vi "Set Result Configuration.vi"(11 "error in (no error)":errorcluster) -> (15 "error out":errorcluster)   [LabVIEW 2021, in "Voltage Measurement.lvlib"]
uses:
  09223ba7-b474-4af4-80b2-5f8b06bdc601.vi
  <vilib>/JDP Science/JSONtext/Variant to JSON Text.vi
  <vilib>/JDP Science/JSONtext/LVClass Serializer/JSONtext LVClass Serializer.lvclass
  Voltage Measurement.lvlib
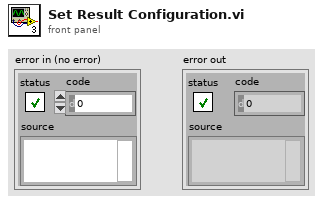
[diagram p1: front panel]
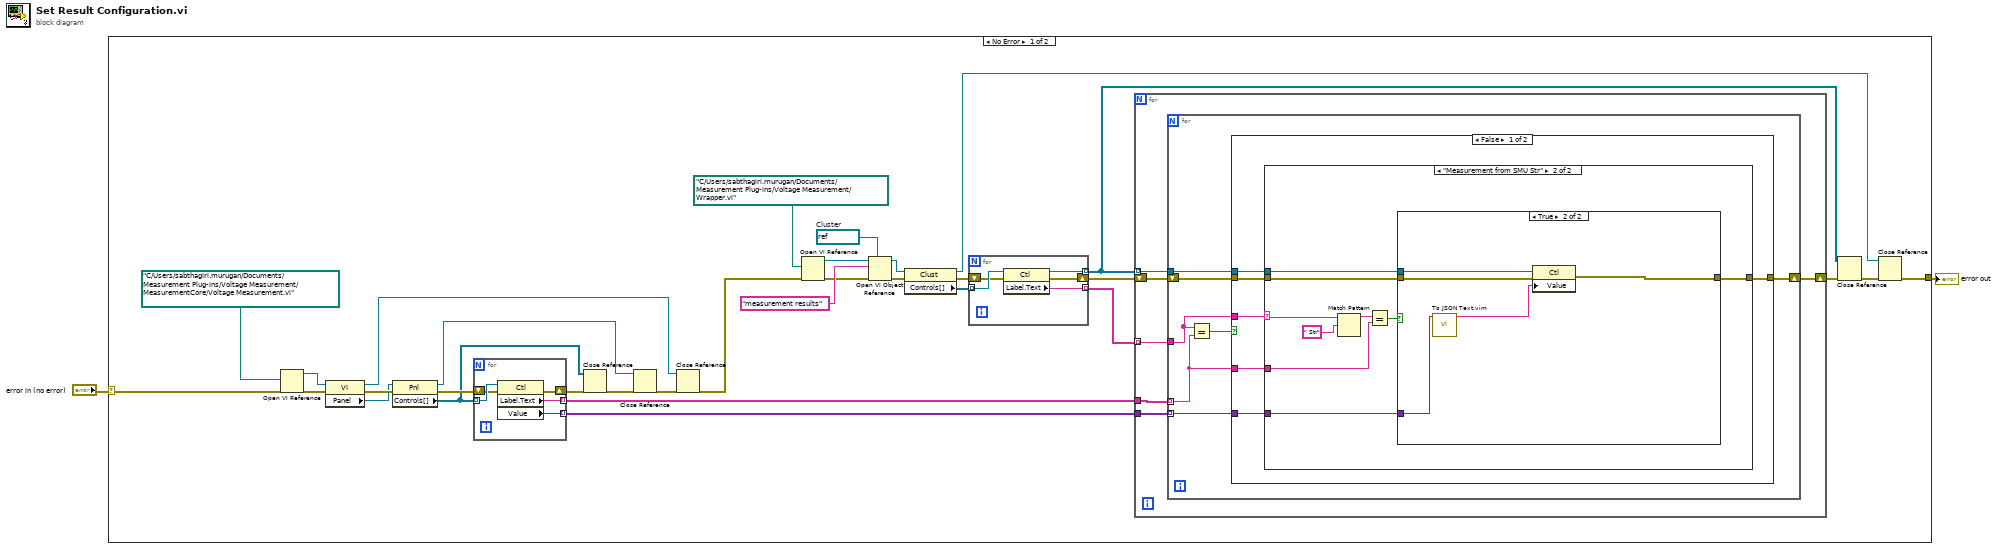
[diagram p0: block diagram]
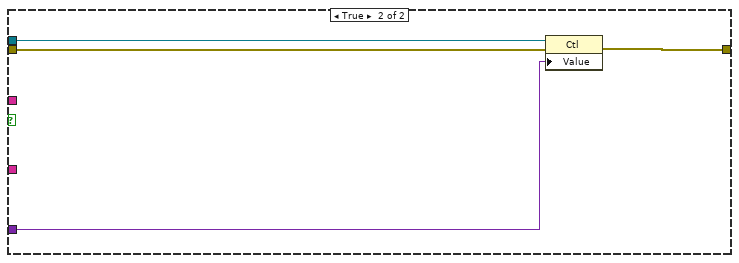
[diagram p4: hidden frame]
diagram:
  n1 = case shown="No Error" "error in (no error)" {
    selector: "error in (no error)" -> [w28 w84]
    tunnel: [w3 w84] -> w2
    frame No Error {
      w22 = refnum<vi> refnum  # Cluster
      n2 = Open VI Reference(vi path=path "C:/Users/sabthagiri.murugan/Documents/Measurement Plug-ins/Voltage Measurement/MeasurementCore/Voltage Measurement.vi", error in (no error)=w28) -> (vi reference=w31:refnum<vi>, error out=w29:errorcluster)  [unwired: 4 in]
      n3 = property class="VI"(reference=w31, error in=w29) -> (reference out=w4:refnum<vi>, error out=w33:errorcluster, "Panel"=w32:refnum<vi>)
      n4 = property class="Pnl"(reference=w32, error in=w33) -> (reference out=w6:refnum<vi>, error out=w34:errorcluster, "Controls[]"=w8:refnum<vi>[])
      n5 = for {
        tunnel: w8 -> [w83] mode=indexing
        shift-right: [w81] -> w17
        shift-left: w34 -> [w82]
        tunnel: [w80] -> w15 mode=indexing
        tunnel: [w79] -> w13 mode=indexing
        n6 = property class="Ctl"(reference=w83, error in=w82) -> (error out=w81:errorcluster, "Label.Text"=w80:string, "Value"=w79:variant)  [unwired: 1 out]
      }
      n7 = Close Reference(reference=w8, error in (no error)=w17) -> (error out=w9:errorcluster)
      n8 = Close Reference(reference=w6, error in (no error)=w9) -> (error out=w7:errorcluster)
      n9 = Close Reference(reference=w4, error in (no error)=w7) -> (error out=w5:errorcluster)
      n10 = Open VI Reference(vi path=path "C:/Users/sabthagiri.murugan/Documents/Measurement Plug-ins/Voltage Measurement/Wrapper.vi", error in (no error)=w5) -> (vi reference=w19:refnum<vi>, error out=w20:errorcluster)  [unwired: 4 in]
      n11 = Open VI Object Reference(7:w22, 8:w20, 10:"measurement results" ("Control Name"), 11:w19) -> (0:w24:errorcluster, 3:w23:refnum<vi>)
      n12 = property class="Clust"(reference=w23, error in=w24) -> (reference out=w27:refnum<vi>, error out=w26:errorcluster, "Controls[]"=w25:refnum<vi>[])
      n13 = for {
        tunnel: w25 -> [w78] mode=indexing
        shift-right: [w76] -> w14
        shift-left: w26 -> [w77]
        tunnel: [w75] -> w16 mode=indexing
        tunnel: [w74] -> w12 mode=indexing
        n14 = property class="Ctl"(reference=w78, error in=w77) -> (reference out=w74:refnum<vi>, error out=w76:errorcluster, "Label.Text"=w75:string)
      }
      n15 = for {
        tunnel: w16 -> [w38] mode=indexing
        tunnel: w12 -> [w37] mode=indexing
        tunnel: w15 -> [w39]
        shift-right: [w35] -> w11
        shift-left: w14 -> [w40]
        tunnel: w13 -> [w36]
        n16 = for {
          shift-right: [w43] -> w35
          shift-left: w40 -> [w47]
          tunnel: w39 -> [w41] mode=indexing
          tunnel: w38 -> [w42]
          tunnel: w37 -> [w45]
          tunnel: w36 -> [w44] mode=indexing
          n17 = Equal?(x=w42, y=w41) -> (x = y?=w46:bool)
          n18 = case shown="False" w46 {
            tunnel: w47 -> [w52 w73]
            tunnel: w45 -> [w51 w72]
            tunnel: w44 -> [w49 w71]
            tunnel: [w48 w70] -> w43
            tunnel: w42 -> [w53 _]
            tunnel: w41 -> [w50 _]
            frame False {
              n19 = case shown="\"Measurement from SMU Str\"" w53 {
                selector: w53 -> [_ w62]
                tunnel: w52 -> [w54 w58]
                tunnel: w51 -> [_ w56]
                tunnel: w50 -> [_ w60]
                tunnel: w49 -> [_ w57]
                tunnel: [w54 w55] -> w48
                frame Default {
                }
                frame "Measurement from SMU Str" {
                  n20 = Match Pattern(string=w62, regular expression=" Str") -> (before substring=w61:string)  [unwired: 1 in, 3 out]
                  n21 = Equal?(x=w61, y=w60) -> (x = y?=w59:bool)
                  n22 = case shown="True" w59 {
                    tunnel: w58 -> [w64 w68]
                    tunnel: w57 -> [_ w69]
                    tunnel: w56 -> [_ w67]
                    tunnel: [w64 w65] -> w55
                    frame False {
                    }
                    frame True {
                      n23 = call "To JSON Text.vim"("Anything"=w69) -> ("<JSON>"=w66:string)  [unwired: 9 in, 1 out]
                      n24 = property class="Ctl"(reference=w67, error in=w68, "Value"=w66) -> (error out=w65:errorcluster)  [unwired: 1 out]
                    }
                  }
                }
              }
            }
            frame True {
              n25 = property class="Ctl"(reference=w72, error in=w73, "Value"=w71) -> (error out=w70:errorcluster)  [unwired: 1 out]
            }
          }
        }
      }
      n26 = Close Reference(reference=w12, error in (no error)=w11) -> (error out=w10:errorcluster)
      n27 = Close Reference(reference=w27, error in (no error)=w10) -> (error out=w3:errorcluster)
    }
    frame Error {
    }
  }
  "error out" <- w2
